vi "Ecrire config Th.vi"(2 "error in (no error)":errorcluster caption="entrée d'erreur (pas d'erreur)", 3 "refnum":T1) -> (0 "error out":errorcluster, 1 "refnum out":T1)   [LabVIEW 2022 SP3]
uses:
  <vilib>/Utility/config.llb/Config Data RefNum.ctl
  Variables globales/Variable glob Th.vi
  <vilib>/Utility/config.llb/Write Key (Boolean).vi
  <vilib>/Utility/config.llb/Write Key (String).vi
  <vilib>/Utility/config.llb/Write Key (U32).vi
  <vilib>/Utility/config.llb/NI_LVConfig.lvlib
panel:
  out "section names":string[](array[string]) caption="noms des sections"
  out "Nb chassis Th":i32
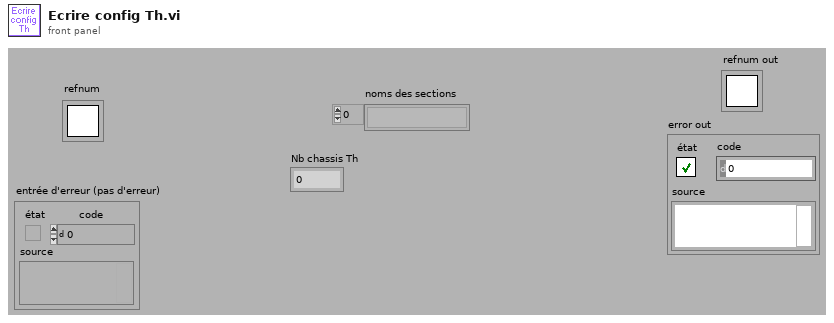
[diagram p1: front panel]
types:
  T1 = typedef "NI_LVConfig.lvlib/Config Data RefNum.ctl" = refnum<k1>
  T2 = cluster{"Nom tache Th":refnum<k21>, "Noms des Th":string[], "Nb Th":i16, "Selection Th":bool[], "Nom Th selectionnes":string[]}[]
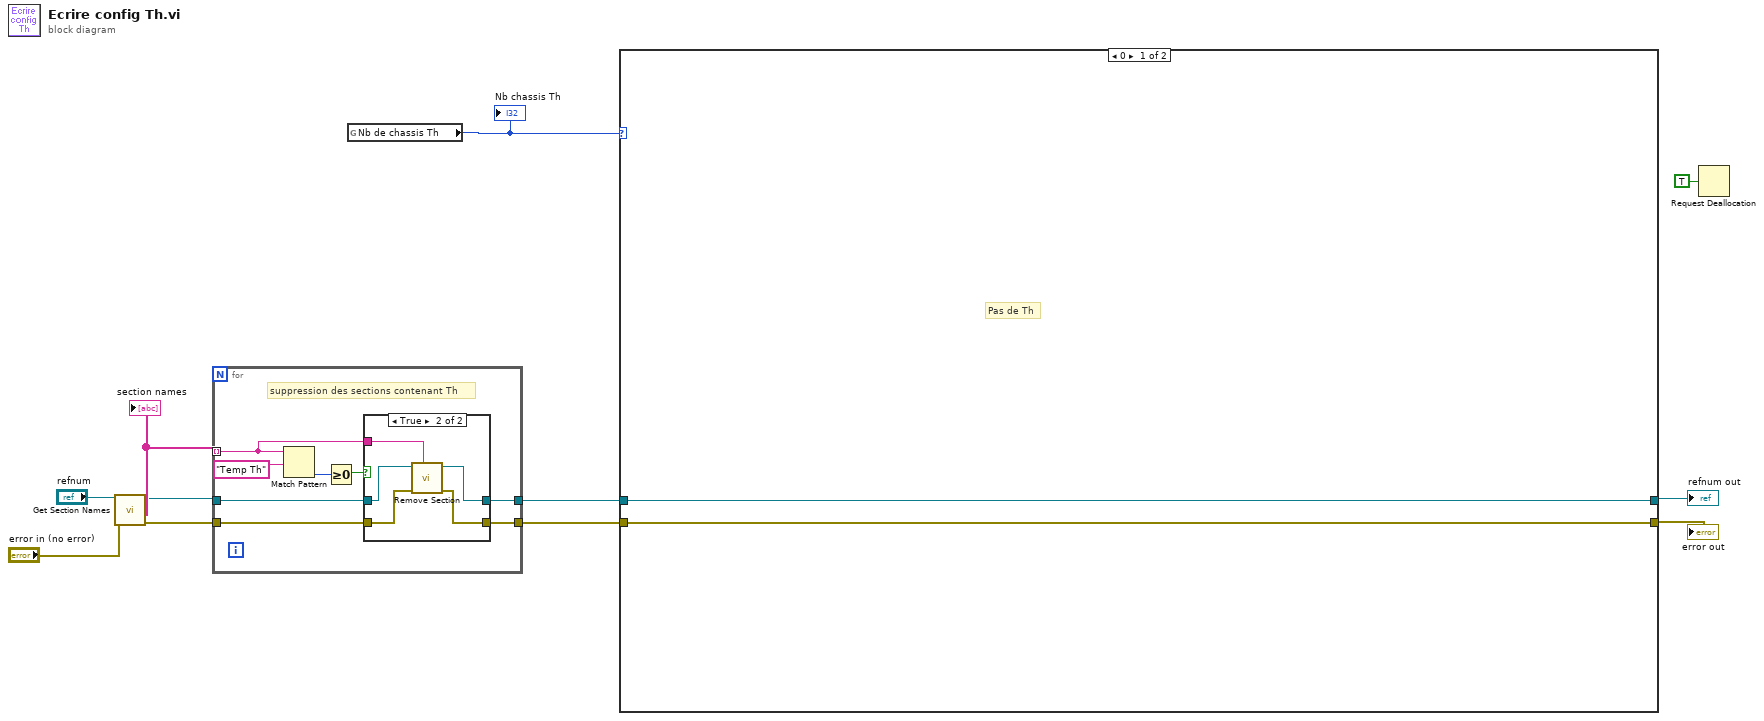
[diagram p0: block diagram]
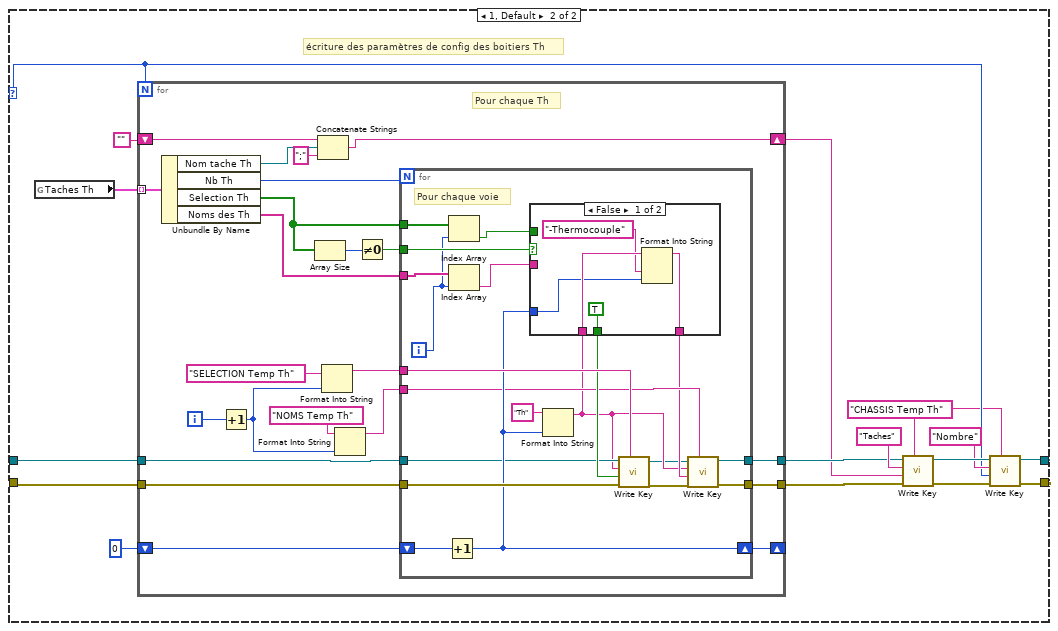
[diagram p2: hidden frame]
diagram:
  n1 = call <vilib>:"Get Section Names.vi"("error in (no error)"="error in (no error)", "refnum"="refnum") -> ("error out"=w8:errorcluster, "section names"=w11:string[], "refnum out"=w9:T1)  [unwired: 7 in]
  "section names" <- w11
  n2 = for {
    tunnel: w11 -> [w16] mode=indexing
    tunnel: w8 -> [w14]
    tunnel: [w12] -> w7
    tunnel: w9 -> [w15]
    tunnel: [w13] -> w10
    # "suppression des sections contenant Th"
    n3 = Match Pattern(string=w16, regular expression="Temp Th" ("expression régulière")) -> (offset past match=w18:i32)  [unwired: 1 in, 3 out]
    n4 = Greater Or Equal To 0?(x=w18) -> (x >= 0?=w17:bool)
    n5 = case shown="True" w17 {
      tunnel: w16 -> [_ w26]
      tunnel: w15 -> [w21 w24]
      tunnel: w14 -> [w20 w25]
      tunnel: [w21 w23] -> w13
      tunnel: [w20 w22] -> w12
      frame False {
      }
      frame True {
        n6 = call <vilib>:"Remove Section.vi"("section"=w26, "error in (no error)"=w25, "refnum"=w24) -> ("error out"=w22:errorcluster, "refnum out"=w23:T1)  [unwired: 6 in, 1 out]
      }
    }
  }
  n7 = global read "Variable glob Th.vi" "Nb de chassis Th"() -> (w2:u8)
  "Nb chassis Th" <- w2
  n8 = case shown="0" w2 {
    selector: w2 -> [_ w40]
    tunnel: w10 -> [w28 w31]
    tunnel: w7 -> [w27 w30]
    tunnel: [w28 w35] -> w4
    tunnel: [w27 w34] -> w3
    frame 0 {
      # "Pas de Th"
    }
    frame 1, Default {
      w38 = "CHASSIS Temp Th" ("section")
      # "écriture des paramètres de config des boitiers Th"
      n9 = global read "Variable glob Th.vi" "Taches Th"() -> (w37:T2)
      n10 = for {
        N: w40 -> [_]
        tunnel: [w63] -> w33
        tunnel: [w62] -> w32
        tunnel: w31 -> [w58]
        tunnel: w30 -> [w57]
        shift-right: [w54] -> _
        shift-left: 0 -> [w55]
        tunnel: w37 -> [w52] mode=indexing
        shift-right: [w45] -> w29
        shift-left: "" -> [w46]
        i -> [w56]
        # "Pour chaque Th"
        n11 = Unbundle By Name(w52) -> ("Nom tache Th"=w47:refnum<k21>, "Nb Th"=w51:i16, "Selection Th"=w50:bool[], "Noms des Th"=w49:string[])
        n12 = Increment(x=w56) -> (x+1=w53:i32)
        n13 = Array Size(array=w50) -> (size(s)=w60:i32)
        n14 = Concatenate Strings(w46, w47, ";" ("chaîne")) -> (w45:string)
        n15 = Format Into String(initial string="SELECTION Temp Th" ("chaîne initiale"), w53) -> (resulting string=w64:string)  [unwired: 2 in, 1 out]
        n16 = Format Into String(initial string="NOMS Temp Th", w53) -> (resulting string=w66:string)  [unwired: 2 in, 1 out]
        n17 = Not Equal To 0?(x=w60) -> (x != 0?=w59:bool)
        n18 = for {
          N: w51 -> [_]
          tunnel: w66 -> [w73]
          tunnel: w64 -> [w85]
          tunnel: w50 -> [w79]
          tunnel: w49 -> [w77]
          tunnel: w59 -> [w81]
          shift-right: [w74] -> w54
          shift-left: w55 -> [w75]
          tunnel: w57 -> [w84]
          tunnel: [w82] -> w62
          tunnel: w58 -> [w72]
          tunnel: [w83] -> w63
          i -> [w70]
          # "Pour chaque voie"
          n19 = Increment(x=w75) -> (x+1=w74:i32)
          n20 = Index Array(array=w79, index=w70) -> (element=w78:bool)
          n21 = Index Array(array=w77, index=w70) -> (element=w76:string)
          n22 = Format Into String(initial string="Th", w74) -> (resulting string=w69:string)  [unwired: 2 in, 1 out]
          n23 = case shown="False" w81 {
            tunnel: w78 -> [_ w93]
            tunnel: w76 -> [_ w92]
            tunnel: [TRUE w93] -> w80
            tunnel: [w90 w92] -> w71
            tunnel: w74 -> [w87 _]
            tunnel: w69 -> [w89 _]
            frame False {
              n24 = Format Into String(initial string=w89, "-Thermocouple" ("chaîne initiale"), w87) -> (resulting string=w90:string)  [unwired: 2 in, 1 out]
            }
            frame True {
            }
          }
          n25 = call-poly <vilib>:"Write Key.vi"("section"=w85, "error in (no error)"=w84, "value"=w80, "key"=w69, "refnum"=w72) -> ("error out"=w67:errorcluster, "refnum out"=w68:T1)  [unwired: 4 in, 1 out]
          n26 = call-poly <vilib>:"Write Key.vi"("section"=w73, "error in (no error)"=w67, "value"=w71, "key"=w69, "refnum"=w68) -> ("error out"=w82:errorcluster, "refnum out"=w83:T1)  [unwired: 4 in, 1 out]
        }
      }
      n27 = call-poly <vilib>:"Write Key.vi"("section"=w38, "error in (no error)"=w32, "value"=w29, "key"="Taches", "refnum"=w33) -> ("error out"=w42:errorcluster, "refnum out"=w43:T1)  [unwired: 4 in, 1 out]
      n28 = call-poly <vilib>:"Write Key.vi"("section"=w38, "error in (no error)"=w42, "value"=w40, "key"="Nombre", "refnum"=w43) -> ("error out"=w34:errorcluster, "refnum out"=w35:T1)  [unwired: 4 in, 1 out]
    }
  }
  "refnum out" <- w4
  "error out" <- w3
  n29 = Request Deallocation(TRUE ("flag")) -> ()
